vi "禁用控件.vi"(6 "控件名称":string[](array[string]), 7 "本VI":refnum<vi>, 8 "错误输入（无错误）":errorcluster, 11 "禁用":T1(ring)) -> (0 "错误输出":errorcluster)   [LabVIEW 2020]
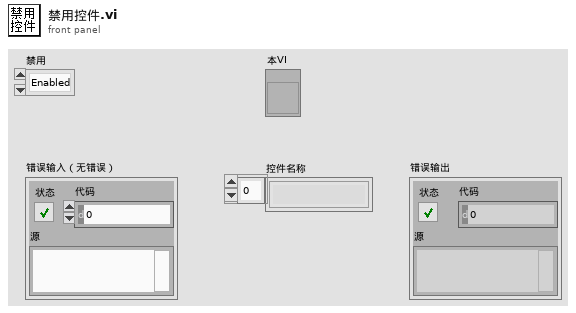
[diagram p1: front panel]
types:
  T1 = enum8{"Enabled", "Disabled", "Disabled and Grayed Out"}
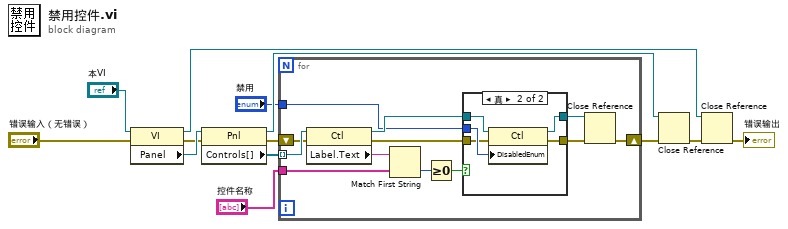
[diagram p0: block diagram]
diagram:
  n1 = property class="VI"(reference="本VI", error in="错误输入（无错误）") -> (reference out=w9:refnum<vi>, error out=w7:errorcluster, "Panel"=w13:refnum<vi>)
  n2 = property class="Pnl"(reference=w13, error in=w7) -> (reference out=w10:refnum<vi>, error out=w6:errorcluster, "Controls[]"=w12:refnum<vi>[])
  n3 = for {
    tunnel: w12 -> [w25] mode=indexing
    tunnel: "禁用" -> [w23]
    shift-right: [w18] -> w5
    shift-left: w6 -> [w21]
    tunnel: "控件名称" -> [w16]
    n4 = property class="Ctl"(reference=w25, error in=w21) -> (reference out=w24:refnum<vi>, error out=w20:errorcluster, "Label.Text"=w17:string)
    n5 = Match First String(2:w16, 3:w17) -> (0:w15:i32)  [unwired: 1 out]
    n6 = Greater Or Equal To 0?(x=w15) -> (x >= 0?=w14:bool)
    n7 = case shown="真" w14 {
      tunnel: w24 -> [w27 w32]
      tunnel: w23 -> [_ w31]
      tunnel: [w27 w30] -> w22
      tunnel: w20 -> [w26 w29]
      tunnel: [w26 w28] -> w19
      frame False {
      }
      frame True {
        n8 = property class="Ctl"(reference=w32, error in=w29, "DisabledEnum"=w31) -> (reference out=w30:refnum<vi>, error out=w28:errorcluster)
      }
    }
    n9 = Close Reference(reference=w22, error in (no error)=w19) -> (error out=w18:errorcluster)
  }
  n10 = Close Reference(reference=w10, error in (no error)=w5) -> (error out=w4:errorcluster)
  n11 = Close Reference(reference=w9, error in (no error)=w4) -> (error out=→"错误输出":errorcluster)
